vi "Tidy Wire Up.vi"(8 "error in (no error)":errorcluster, 9 "Remove Loose Ends":bool=TRUE, 10 "Clean up Wire":bool=TRUE, 11 "Wire":refnum<vi>) -> (0 "error out":errorcluster, 3 "Out":refnum<vi>)   [LabVIEW 2012, in "Scripting Tools.lvlib"]
uses:
  <userlib>/_LAVAcr/Scripting Tools/Scripting Tools.lvlib
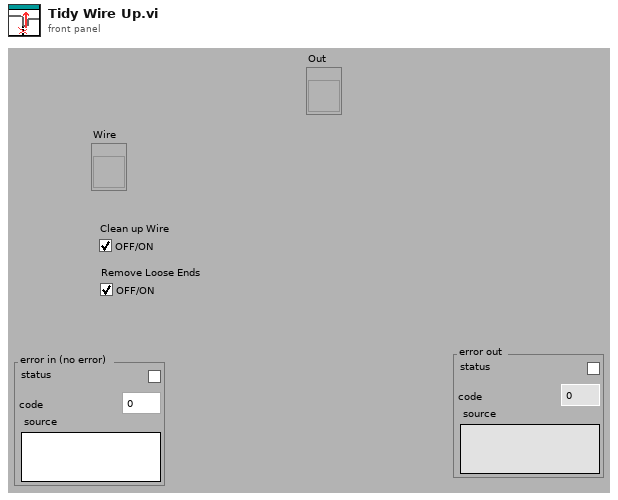
[diagram p1: front panel]
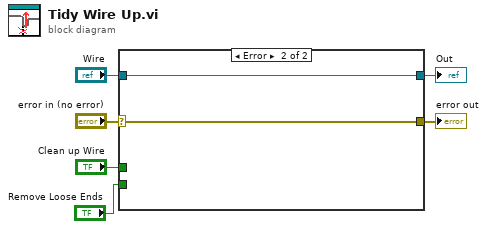
[diagram p0: block diagram]
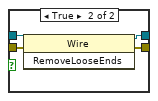
[diagram p3: hidden frame]
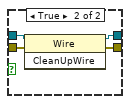
[diagram p4: hidden frame]
diagram:
  n1 = case shown="Error" "error in (no error)" {
    selector: "error in (no error)" -> [w13 w28]
    tunnel: "Clean up Wire" -> [w14 _]
    tunnel: "Wire" -> [w12 w27]
    tunnel: "Remove Loose Ends" -> [w11 _]
    tunnel: [w8 w28] -> w2
    tunnel: [w7 w27] -> w1
    frame No Error {
      n2 = case shown="False" w14 {
        tunnel: w13 -> [w22 w26]
        tunnel: w12 -> [w21 w25]
        tunnel: [w22 w24] -> w10
        tunnel: [w21 w23] -> w9
        frame False {
        }
        frame True {
          n3 = invoke class="Wire" method="CleanUpWire"(reference=w25, error in=w26) -> (reference out=w23:refnum<vi>, error out=w24:errorcluster)  [unwired: 1 in, 1 out]
        }
      }
      n4 = case shown="False" w11 {
        tunnel: w10 -> [w16 w20]
        tunnel: w9 -> [w15 w19]
        tunnel: [w16 w18] -> w8
        tunnel: [w15 w17] -> w7
        frame False {
        }
        frame True {
          n5 = invoke class="Wire" method="RemoveLooseEnds"(reference=w19, error in=w20) -> (reference out=w17:refnum<vi>, error out=w18:errorcluster)  [unwired: 1 in, 1 out]
        }
      }
    }
    frame Error {
    }
  }
  "error out" <- w2
  "Out" <- w1
